vi "available tag dialog.vi"(6 "Call Back VI":T1, 7 "channel action event":refnum<user-event>, 8 "error in":errorcluster, 10 "channel to map to":refnum<class "TBM channel.lvclass">, 11 "filtered tags":refnum<class "tag descriptor.lvclass">[](array[class])) -> (0 "error out":errorcluster)   [LabVIEW 2013, in "Table Manager.lvlib"]
uses:
  Table Manager.lvlib
  <vilib>/NI/Tag Bus/tag/tag descriptor.lvclass
  channel action event.ctl
  dialog output action.ctl
  <vilib>/NI/Tag Bus Module Framework/channel/TBM channel.lvclass
  Table Manager/Call Back Ref Type Def.ctl
  Configuration Editor/Classes/Engine Parent/Engine Parent Editor Node.lvclass
  Configuration Editor/Classes/Module editor node/module editor node.lvclass
  <vilib>/event_ctls.llb/usereventprio.ctl
  <vilib>/NI/Tag Bus/tag/tag descriptor.lvclass/tag descriptor.ctl
  Table Manager/Table Manager.lvclass
panel:
  in  "Set Default":bool
  in  "Create Tag":bool
  in  "Filter":string
  in  "Available Tags":i32(listbox)
  in  "disconnect":bool
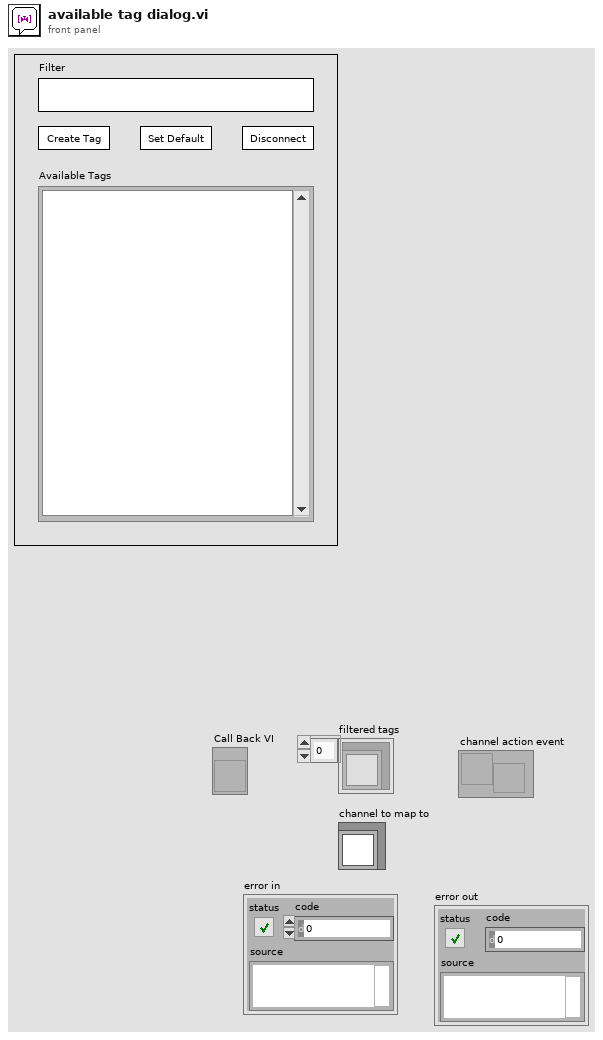
[diagram p1: front panel]
types:
  T1 = typedef "Table Manager.lvlib/Table Manager.lvclass/Call Back Ref Type Def.ctl" = refnum<vi>
  T2 = typedef "usereventprio.ctl" = enum32{"high priority", "normal priority"}
  T3 = typedef "Table Manager.lvlib/dialog output action.ctl" = enum16{"Tag Created", "Tag Selected", "Set Default", "disconnect"}
  T4 = typedef "Table Manager.lvlib/channel action event.ctl" = cluster{"action":T3, "channel":refnum<class "TBM channel.lvclass">, "selected tag":refnum<class "tag descriptor.lvclass">, "Call Back VI":T1}
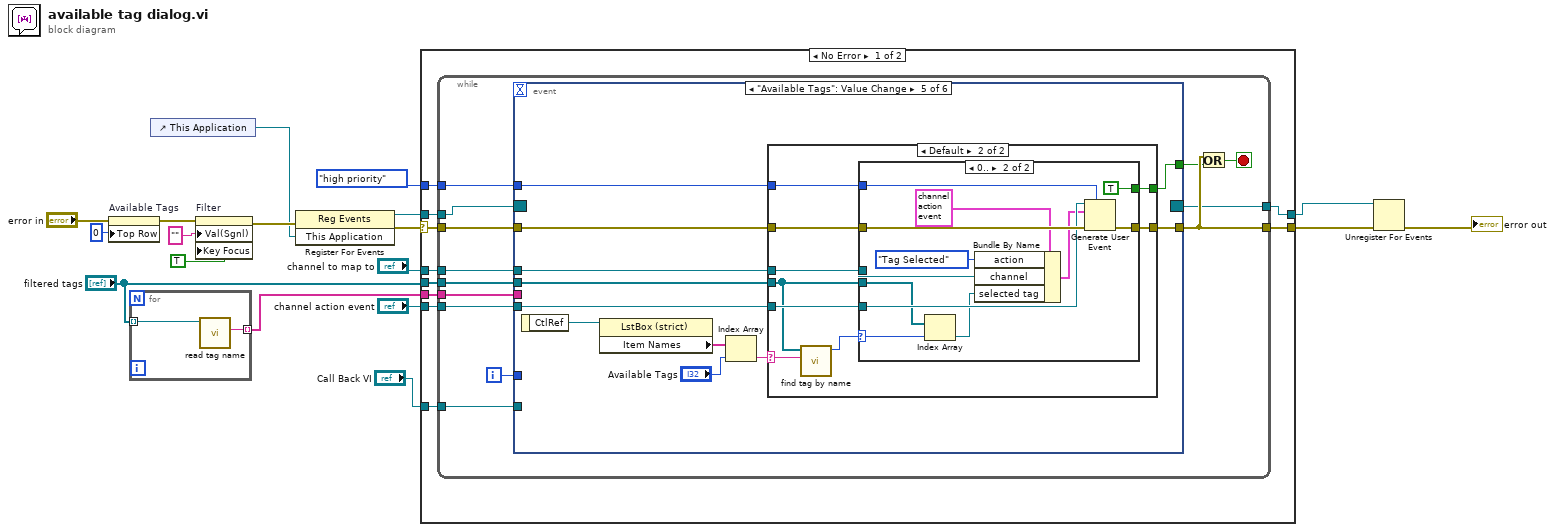
[diagram p0: block diagram]
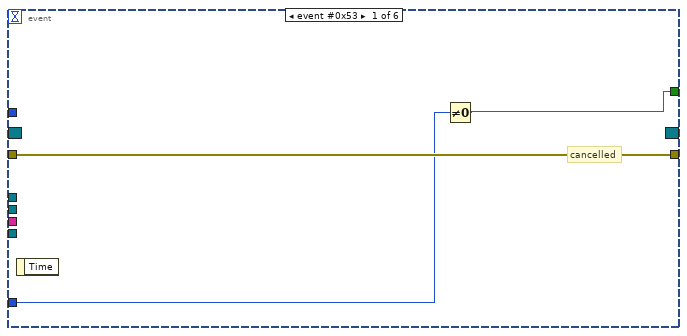
[diagram p2: hidden frame]
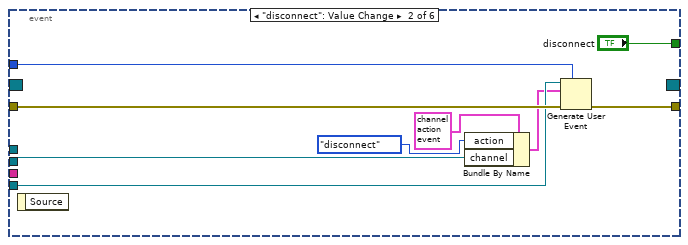
[diagram p3: hidden frame]
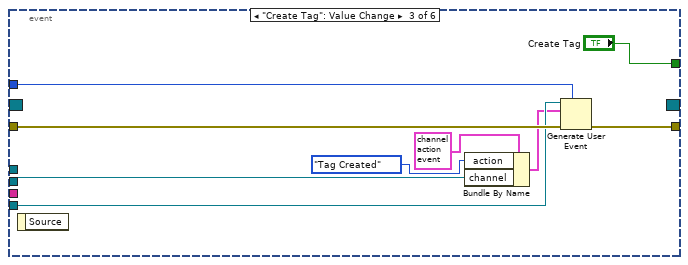
[diagram p4: hidden frame]
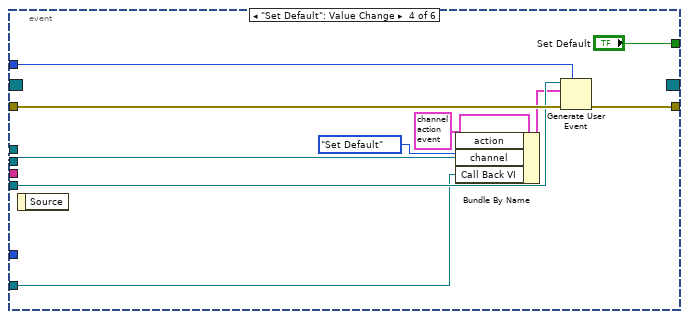
[diagram p5: hidden frame]
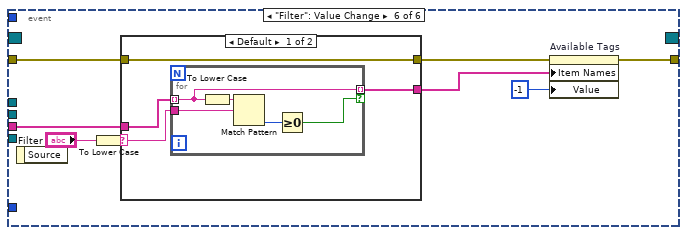
[diagram p8: hidden frame]
diagram:
  n1 = property on="Available Tags" class="LstBox (strict)"(error in="error in", "Top Row"=0) -> (error out=w2:errorcluster)  [unwired: 1 in, 1 out]
  n2 = for {
    tunnel: "filtered tags" -> [w20] mode=indexing
    tunnel: [w19] -> w13 mode=indexing
    n3 = call <vilib>:"read tag name.vi"("system tag in"=w20) -> ("name"=w19:string)  [unwired: 8 in, 2 out]
  }
  n4 = control-ref of="This Application"() -> (w5:refnum<vi>)
  n5 = property on="Filter" class="Str"(error in=w2, "Val(Sgnl)"="" ("Value (Signaling)"), "Key Focus"=TRUE) -> (error out=w12:errorcluster)  [unwired: 1 in, 1 out]
  n6 = register-events(error in=w12, w5) -> (reference out=w8:refnum<event-registration>, error out=w9:errorcluster)  [unwired: 1 in]
  n7 = case shown="No Error" w9 {
    selector: w9 -> [w28 w129]
    tunnel: [w30 w129] -> w18
    tunnel: "channel action event" -> [w29 _]
    tunnel: "channel to map to" -> [w27 _]
    tunnel: usereventprio."high priority" ("priority (normal)") -> [w26 _]
    tunnel: "filtered tags" -> [w25 _]
    tunnel: w13 -> [w24 _]
    tunnel: w8 -> [w23 w128]
    tunnel: [w22 w128] -> w6
    tunnel: "Call Back VI" -> [w21 _]
    frame No Error {
      n8 = while {
        tunnel: w28 -> [w43]
        tunnel: [w41] -> w30
        tunnel: w29 -> [w39]
        tunnel: w27 -> [w38]
        tunnel: w26 -> [w37]
        tunnel: w25 -> [w36]
        tunnel: w24 -> [w35]
        tunnel: w23 -> [w33]
        tunnel: [w32] -> w22
        tunnel: w21 -> [w31]
        i -> [w34]
        stop <- w42 stop-if-true
        n9 = event shown="[4] \"Available Tags\": Value Change" {
          selector: w33 -> [_ _ _ _ _ _]
          dyn-events: [_ _ _ _ _ _] -> w32
          timeout: _ -> [_ _ _ _ _ _]
          tunnel: w43 -> [w46 w55 w64 w74 w85 w116]
          tunnel: [w46 w54 w63 w73 w84 w113] -> w41
          tunnel: [w45 "disconnect" "Create Tag" "Set Default" w76 _] -> w40
          tunnel: w39 -> [_ w53 w62 w72 w83 _]
          tunnel: w38 -> [_ w49 w58 w68 w82 _]
          tunnel: w37 -> [_ w48 w57 w67 w81 _]
          tunnel: w36 -> [_ _ _ _ w77 _]
          tunnel: w35 -> [_ _ _ _ _ w110]
          tunnel: w34 -> [w44 _ _ _ _ _]
          tunnel: w31 -> [_ _ _ w65 _ _]
          event event #0x53 {
            # "cancelled"
            n10 = event-data() -> ()  [unwired: 1 in, 1 out]
            n11 = Not Equal To 0?(x=w44) -> (x != 0?=w45:bool)
          }
          event "disconnect": Value Change {
            n12 = event-data() -> ()  [unwired: 1 in, 1 out]
            n13 = Bundle By Name(cluster=T4 {"action"=enum."Tag Created", "channel"=refnum, "selected tag"=refnum, "Call Back VI"=refnum} ("event data"), "action"=dialog_output_action."disconnect", "channel"=w49) -> (w51:T4)
            n14 = Generate User Event(priority (normal)=w48, user event=w53, event data cluster=w51, error in=w55) -> (error out=w54:errorcluster)  [unwired: 1 out]
          }
          event "Create Tag": Value Change {
            n15 = event-data() -> ()  [unwired: 1 in, 1 out]
            n16 = Bundle By Name(cluster=T4 {"action"=enum."Tag Created", "channel"=refnum, "selected tag"=refnum, "Call Back VI"=refnum} ("event data"), "action"=dialog_output_action."Tag Created", "channel"=w58) -> (w60:T4)
            n17 = Generate User Event(priority (normal)=w57, user event=w62, event data cluster=w60, error in=w64) -> (error out=w63:errorcluster)  [unwired: 1 out]
          }
          event "Set Default": Value Change {
            n18 = event-data() -> ()  [unwired: 1 in, 1 out]
            n19 = Bundle By Name(cluster=T4 {"action"=enum."Tag Created", "channel"=refnum, "selected tag"=refnum, "Call Back VI"=refnum} ("event data"), "action"=dialog_output_action."Set Default", "channel"=w68, "Call Back VI"=w65) -> (w70:T4)
            n20 = Generate User Event(priority (normal)=w67, user event=w72, event data cluster=w70, error in=w74) -> (error out=w73:errorcluster)  [unwired: 1 out]
          }
          event "Available Tags": Value Change {
            n21 = event-data() -> ("CtlRef"=w80:refnum<vi>)  [unwired: 1 in]
            n22 = property class="LstBox (strict)"(reference=w80) -> ("Item Names"=w79:string[])  [unwired: 1 in, 2 out]
            n23 = Index Array(array=w79, index="Available Tags") -> (element=w78:string)
            n24 = case shown="Default" w78 {
              selector: w78 -> [_ w90]
              tunnel: w85 -> [w86 w95]
              tunnel: [w86 w94] -> w84
              tunnel: w83 -> [_ w93]
              tunnel: w82 -> [_ w92]
              tunnel: w81 -> [_ w91]
              tunnel: w77 -> [_ w88]
              tunnel: [_ w87] -> w76
              frame "" {
              }
              frame Default {
                n25 = call <vilib>:"find tag by name.vi"("name"=w90, "tags in"=w88) -> ("index"=w89:i32)  [unwired: 9 in]
                n26 = case shown="0.." w89 {
                  selector: w89 -> [_ w100]
                  tunnel: w95 -> [w96 w108]
                  tunnel: [w96 w107] -> w94
                  tunnel: w93 -> [_ w106]
                  tunnel: w92 -> [_ w102]
                  tunnel: w91 -> [_ w101]
                  tunnel: w88 -> [_ w99]
                  tunnel: [_ TRUE] -> w87
                  frame ..-1 {
                  }
                  frame 0.. {
                    n27 = Index Array(array=w99, index=w100) -> (element=w98:refnum<class "tag descriptor.lvclass">)
                    n28 = Bundle By Name(cluster=T4 {"action"=enum."Tag Created", "channel"=refnum, "selected tag"=refnum, "Call Back VI"=refnum} ("event data"), "action"=dialog_output_action."Tag Selected", "channel"=w102, "selected tag"=w98) -> (w104:T4)
                    n29 = Generate User Event(priority (normal)=w101, user event=w106, event data cluster=w104, error in=w108) -> (error out=w107:errorcluster)  [unwired: 1 out]
                  }
                }
              }
            }
          }
          event "Filter": Value Change {
            n30 = event-data() -> ()  [unwired: 1 in, 1 out]
            n31 = To Lower Case(string="Filter") -> (all lower case string=w109:string)
            n32 = case shown="Default" w109 {
              selector: w109 -> [w119 _]
              tunnel: w116 -> [w120 w127]
              tunnel: [w120 w127] -> w112
              tunnel: [w117 w126] -> w111
              tunnel: w110 -> [w118 w126]
              frame Default {
                n33 = for {
                  tunnel: w119 -> [w125]
                  tunnel: w118 -> [w124] mode=indexing
                  tunnel: [w124] -> w117 mode=indexing if=w122
                  n34 = To Lower Case(string=w124) -> (all lower case string=w121:string)
                  n35 = Match Pattern(string=w121, regular expression=w125) -> (offset past match=w123:i32)  [unwired: 1 in, 3 out]
                  n36 = Greater Or Equal To 0?(x=w123) -> (x >= 0?=w122:bool)
                }
              }
              frame "" {
              }
            }
            n37 = property on="Available Tags" class="LstBox (strict)"(error in=w112, "Item Names"=w111, "Value"=-1 ("Available Tags")) -> (error out=w113:errorcluster)  [unwired: 1 in, 1 out]
          }
        }
        n38 = Or(x=w41, y=w40) -> (x .or. y?=w42:bool)
      }
    }
    frame Error {
    }
  }
  n39 = Unregister For Events(event registration refnum=w6, error in=w18) -> (error out=→"error out":errorcluster)
